vi "Test Server Restart While Client Retries.vi"(8 "error in (no error)":errorcluster) -> (0 "error out":errorcluster)   [LabVIEW 2019, in "RemoteControl.ZMQ.Tests.lvclass"]
uses:
  RemoteControl.ZMQ.Tests.lvclass
  C:/Program Files/National Instruments/LabVIEW 2019/user.lib/LevyLab/RemoteControl/RemoteControl/RemoteControl.lvclass
  <userlib>/LevyLab/RemoteControl/RemoteControl/RemoteControl.lvclass/RemoteControl.ctl
  <vilib>/numeric/Random Number (Range) U64.vi
  f0f0e852-f0d2-4d3c-8996-27ebcacf9f61.vi
  <vilib>/numeric/sub_Random U32.vi
  f0f0e852-f0d2-4d3c-8996-27ebcacf9f61.vi/7c99dda3-071f-4f08-9a2c-ab661024165e.vi
  f0f0e852-f0d2-4d3c-8996-27ebcacf9f61.vi/57197ae9-7ae2-447f-86de-9249130d4f3d.vi
  <vilib>/Utility/Data Type/Get Type Information.vi
  <vilib>/JDP Science/JSONtext/JSON text to Variant.vi
  <vilib>/addons/_JKI Toolkits/Caraya/classes/Assert/Assert True.vi
  <vilib>/JDP Science/JSONtext/LVClass Serializer/JSONtext LVClass Serializer.lvclass
  <userlib>/LevyLab/RemoteControl/RemoteControl/RemoteControl.lvclass
  <vilib>/addons/_JKI Toolkits/Caraya/classes/Assert/Assert.lvclass
  <vilib>/addons/_JKI Toolkits/Caraya/classes/Test/Test.lvclass
panel:
  out "min time (ms)":u32
  out "max time (ms)":u32
  out "Equal?":bool[](array[boolean])
  out "Codes":i32[](array[numeric])
  in  "stop":bool
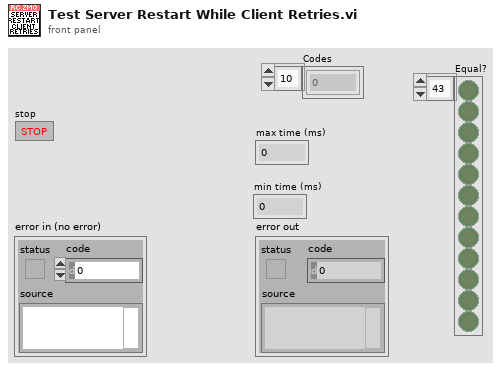
[diagram p1: front panel]
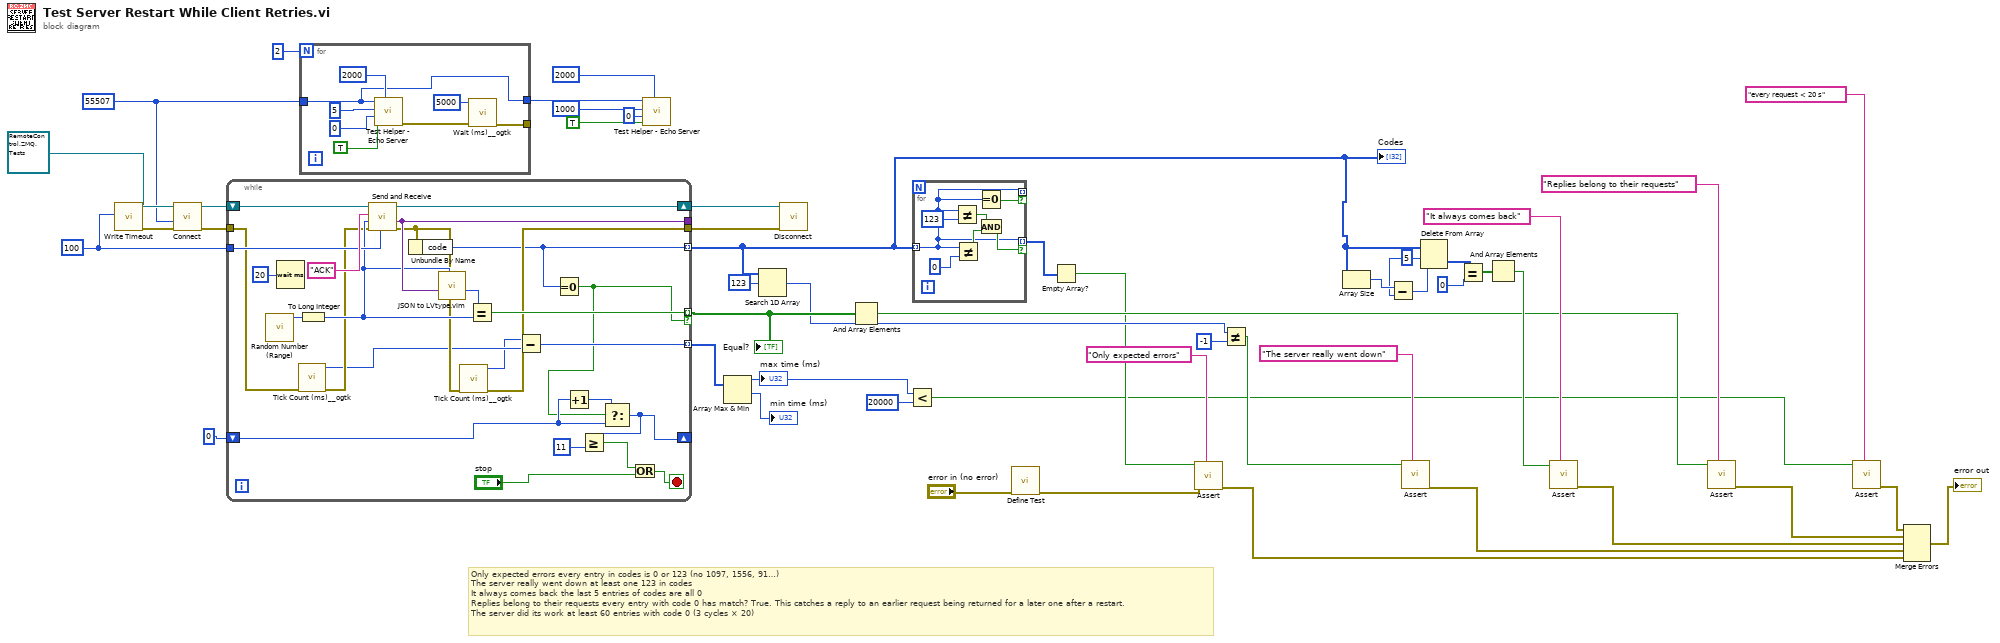
[diagram p0: block diagram]
diagram:
  w22 = 5 ("length")
  w40 = 100 ("timeout in ms (100)")
  w11 = u16 55507 ("Port")
  # "Only expected errors\tevery entry in codes is 0 or 123 (no 1097, 1556, 91…)\nThe server really went down\tat least one 123 in codes\nIt always comes back\tthe last 5 entries of codes are all 0\nReplies belong to their requests\tevery entry with code 0 has match? True. This catches a reply to an earlier request being returned for a later one after a restart.\nThe server did its work\tat least 60 entries with code 0 (3 cycles × 20)"
  n1 = call <userlib>:"Write Timeout.vi"("timeout (ms) [500]"=w40, "RemoteControl in"=refnum<class "RemoteControl.ZMQ.Tests.lvclass"> refnum ("RemoteControl.ZMQ.Tests.lvclass")) -> ("error out"=w43:errorcluster, "RemoteControl out"=w42:refnum<class "RemoteControl.ZMQ.Tests.lvclass">)  [unwired: 8 in]
  n2 = call <userlib>:"Connect.vi"("error in (no error)"=w43, "Port"=w11, "RemoteControl in"=w42) -> ("error out"=w48:errorcluster, "RemoteControl out"=w50:refnum<class "RemoteControl.ZMQ.Tests.lvclass">)  [unwired: 7 in]
  n3 = while {
    tunnel: [w71] -> _
    tunnel: w40 -> [w72]
    shift-right: [w75] -> w49
    shift-left: w50 -> [w76]
    tunnel: w48 -> [w65]
    tunnel: [w63] -> w47
    tunnel: [w57] -> w20 mode=indexing
    tunnel: [w68] -> w33 mode=indexing if=w53
    tunnel: [w61] -> w6 mode=indexing
    shift-right: [w52] -> _
    shift-left: 0 ("milliseconds to wait") -> [w54]
    stop <- w58 stop-if-true
    n4 = call-poly <vilib>:"Random Number (Range).vi"() -> ("number"=w74:u64)  [unwired: 11 in]
    n5 = Wait (ms)(milliseconds to wait=u32 20) -> ()  [unwired: 1 out]
    n6 = call <userlib>:"Tick Count (ms)__ogtk.vi"("error in (no error)"=w65) -> ("error out"=w66:errorcluster, "millisecond timer value"=w62:u32)  [unwired: 9 in]
    n7 = To Long Integer(number=w74) -> (32bit integer=w69:i32)
    n8 = call <userlib>:"Send and Receive.vi"("timeout (ms) [500]"=w72, "error in (no error)"=w66, "Data"=w69, "Command"="ACK", "RemoteControl in"=w76) -> ("error out"=w64:errorcluster, "Data out"=w71:variant, "RemoteControl out"=w75:refnum<class "RemoteControl.ZMQ.Tests.lvclass">)  [unwired: 3 in, 1 out]
    n9 = Unbundle By Name(w64) -> ("code"=w57:i32)
    n10 = call "JSON to LVtype.vim"("type"=w69, "JSON Data in"=w71) -> ("Data out"=w70:i32)  [unwired: 8 in, 1 out]
    n11 = call <userlib>:"Tick Count (ms)__ogtk.vi"("error in (no error)"=w64) -> ("error out"=w63:errorcluster, "millisecond timer value"=w60:u32)  [unwired: 9 in]
    n12 = Equal?(x=w70, y=w69) -> (x = y?=w68:bool)
    n13 = Subtract(x=w60, y=w62) -> (x-y=w61:u32)
    n14 = Equal To 0?(x=w57) -> (x = 0?=w53:bool)
    n15 = Increment(x=w54) -> (x+1=w56:i32)
    n16 = Select(t=w56, s=w53, f=w54) -> (s? t:f=w52:i32)
    n17 = Greater Or Equal?(x=w52, y=11) -> (x >= y?=w51:bool)
    n18 = Or(x=w51, y="stop") -> (x .or. y?=w58:bool)
  }
  "Codes" <- w20
  "Equal?" <- w33
  n19 = for {
    N: 2 -> [_]
    tunnel: w11 -> [w77]
    tunnel: [w79] -> _
    tunnel: [w77] -> w8
    n20 = call "Test Helper - Echo Server.vi"("idle timout"=u32 2000, "Answer?"=TRUE, "reply delay (ms)"=u32 0, "number of messages"=5, "port"=w77) -> ("error out"=w81:errorcluster)  [unwired: 5 in, 1 out]
    n21 = call <userlib>:"Wait (ms)__ogtk.vi"("error in (no error)"=w81, "milliseconds to wait"=u32 5000) -> ("error out"=w79:errorcluster)  [unwired: 8 in, 1 out]
  }
  n22 = call "Test Helper - Echo Server.vi"("idle timout"=u32 2000, "Answer?"=TRUE, "reply delay (ms)"=u32 0, "number of messages"=1000, "port"=w8) -> ()  [unwired: 5 in, 2 out]
  n23 = Array Max & Min(array=w6) -> (max value=w4:u32, min value=→"min time (ms)":u32)  [unwired: 2 out]
  "max time (ms)" <- w4
  n24 = Search 1D Array(1D array=w20, element=123) -> (index of element=w26:i32)  [unwired: 1 in]
  n25 = call <userlib>:"Disconnect.vi"("error in (no error)"=w47, "RemoteControl in"=w49) -> ()  [unwired: 8 in, 2 out]
  n26 = And Array Elements(Boolean array=w33) -> (logical AND=w32:bool)
  n27 = Less?(x=w4, y=u32 20000) -> (x < y?=w3:bool)
  n28 = for {
    tunnel: w20 -> [w86] mode=indexing
    tunnel: [w86] -> w28 mode=indexing if=w87
    tunnel: [w86] -> _ mode=indexing if=w85
    n29 = Not Equal?(x=w86, y=123) -> (x != y?=w89:bool)
    n30 = Not Equal?(x=w86, y=0) -> (x != y?=w88:bool)
    n31 = Equal To 0?(x=w86) -> (x = 0?=w85:bool)
    n32 = And(x=w89, y=w88) -> (x .and. y?=w87:bool)
  }
  n33 = call <vilib>:"Define Test.vi"("error in (no error)"="error in (no error)") -> ("error out"=w19:errorcluster)  [unwired: 9 in, 1 out]
  n34 = Empty Array?(array=w28) -> (empty?=w25:bool)
  n35 = call-poly <vilib>:"Assert.vi"("Label"="Only expected errors", "error in (no error)"=w19, "True?"=w25) -> ("error out"=w14:errorcluster)  [unwired: 7 in, 1 out]
  n36 = Not Equal?(x=w26, y=-1) -> (x != y?=w29:bool)
  n37 = Array Size(array=w20) -> (size(s)=w23:i32)
  n38 = Subtract(x=w23, y=w22) -> (x-y=w21:i32)
  n39 = call-poly <vilib>:"Assert.vi"("Label"="The server really went down", "True?"=w29) -> ("error out"=w15:errorcluster)  [unwired: 8 in, 1 out]
  n40 = Delete From Array(array=w20, length=w22, index=w21) -> (deleted portion=w37:i32[])  [unwired: 1 out]
  n41 = Equal?(x=w37, y=0 ("length")) -> (x = y?=w35:bool[])
  n42 = And Array Elements(Boolean array=w35) -> (logical AND=w34:bool)
  n43 = call-poly <vilib>:"Assert.vi"("Label"="It always comes back", "True?"=w34) -> ("error out"=w16:errorcluster)  [unwired: 8 in, 1 out]
  n44 = call-poly <vilib>:"Assert.vi"("Label"="Replies belong to their requests", "True?"=w32) -> ("error out"=w17:errorcluster)  [unwired: 8 in, 1 out]
  n45 = call-poly <vilib>:"Assert.vi"("Label"="every request < 20 s", "True?"=w3) -> ("error out"=w18:errorcluster)  [unwired: 8 in, 1 out]
  n46 = Merge Errors(w18, w17, w16, w15, w14) -> (→"error out":errorcluster)
